vi "4.2 Arguments - Error As Arguments.vi"() -> ()   [LabVIEW 2017]
doc: "#### Overview\n\nThis example demonstrates how LabVIEW errors are passed as CSM arguments.\n\n#### Introduction\n\nThis example converts a LabVIEW error cluster into a CSM-compatible error string. This allows the CSM core parsing engine to handle LabVIEW errors from the message queue and facilitates logging internal errors. The converted error string uses the following format: `<ErrStr>[Error: error-code] error-description-As-safe-argument-string`. Additionally, `CSM - Argument Type.vi` retrieves the argument tag, which in this case is `ErrStr`.\n\n<b>Application Scenario</b>: Passing LabVIEW errors.\n\n#### Steps\n\n- Step1: Demonstrate converting an error to ErrStr and restoring it.\n- Step2: (Forward Compatibility) Demonstrate converting a previous ErrStr back to an error cluster.\n- Step3: Demonstrate converting a previous ErrStr back to an error cluster and obtaining the CSM-Argument Type."
uses:
  user.lib/_NEVSTOP/Communicable State Machine(CSM)/AdvanceAPI/CSM - Revert Arguments-Safe String.vi
  user.lib/_NEVSTOP/Communicable State Machine(CSM)/AdvanceAPI/CSM - Make String Arguments Safe.vi
  user.lib/_NEVSTOP/Communicable State Machine(CSM)/AdvanceAPI/CSM - Keywords.vi
  user.lib/_NEVSTOP/Communicable State Machine(CSM)/_Shared/Trim Single-line Text.vi
  user.lib/_NEVSTOP/Communicable State Machine(CSM)/Communicable State Machine.lvlib
  user.lib/_NEVSTOP/Communicable State Machine(CSM)/_Shared/CSM Shared.lvlib
panel:
  out "error 2":errorcluster
  out "Warning Arguments":string
  out "argument token":string
  out "<ErrStr>[Error: 472]Error String 1%0AError String 2%0AError String 3":errorcluster
  out "[Error: 502]Error String 1%0AError String 2%0AError String 3":errorcluster
  out "Error Arguments":string
  out "error":errorcluster
  # "#CSM-Example Overview\n\nThis example demonstrates how LabVIEW errors are passed as CSM arguments."
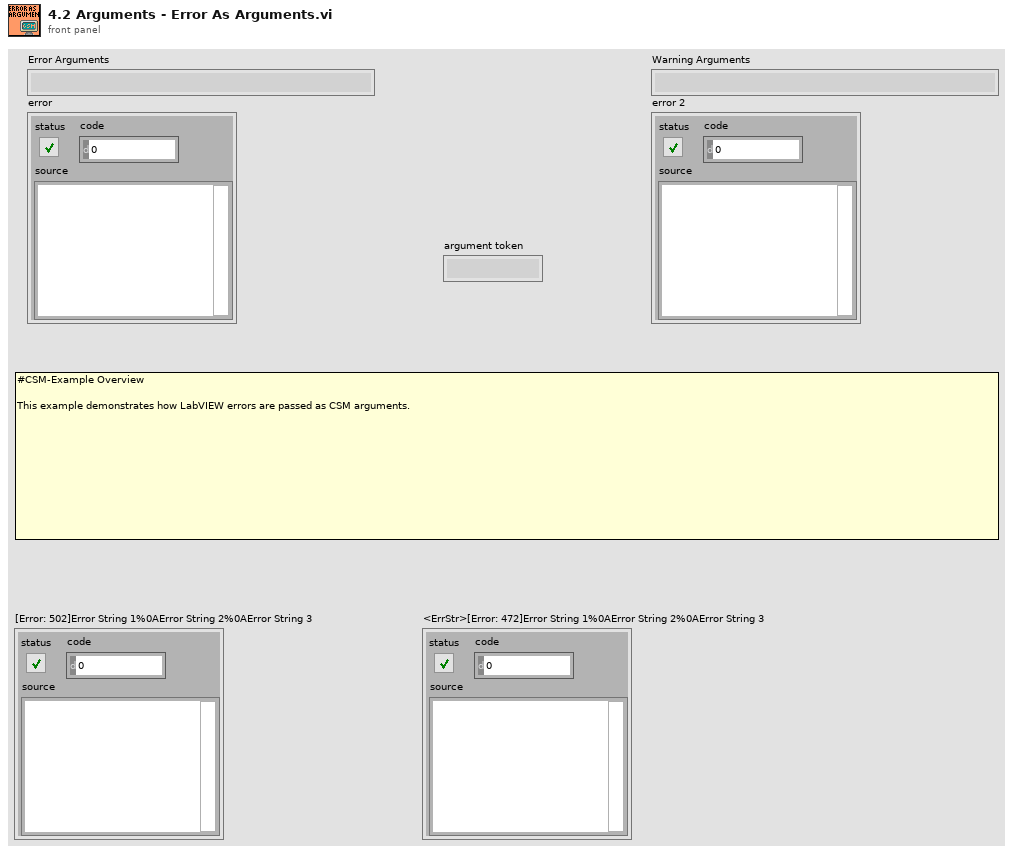
[diagram p1: front panel]
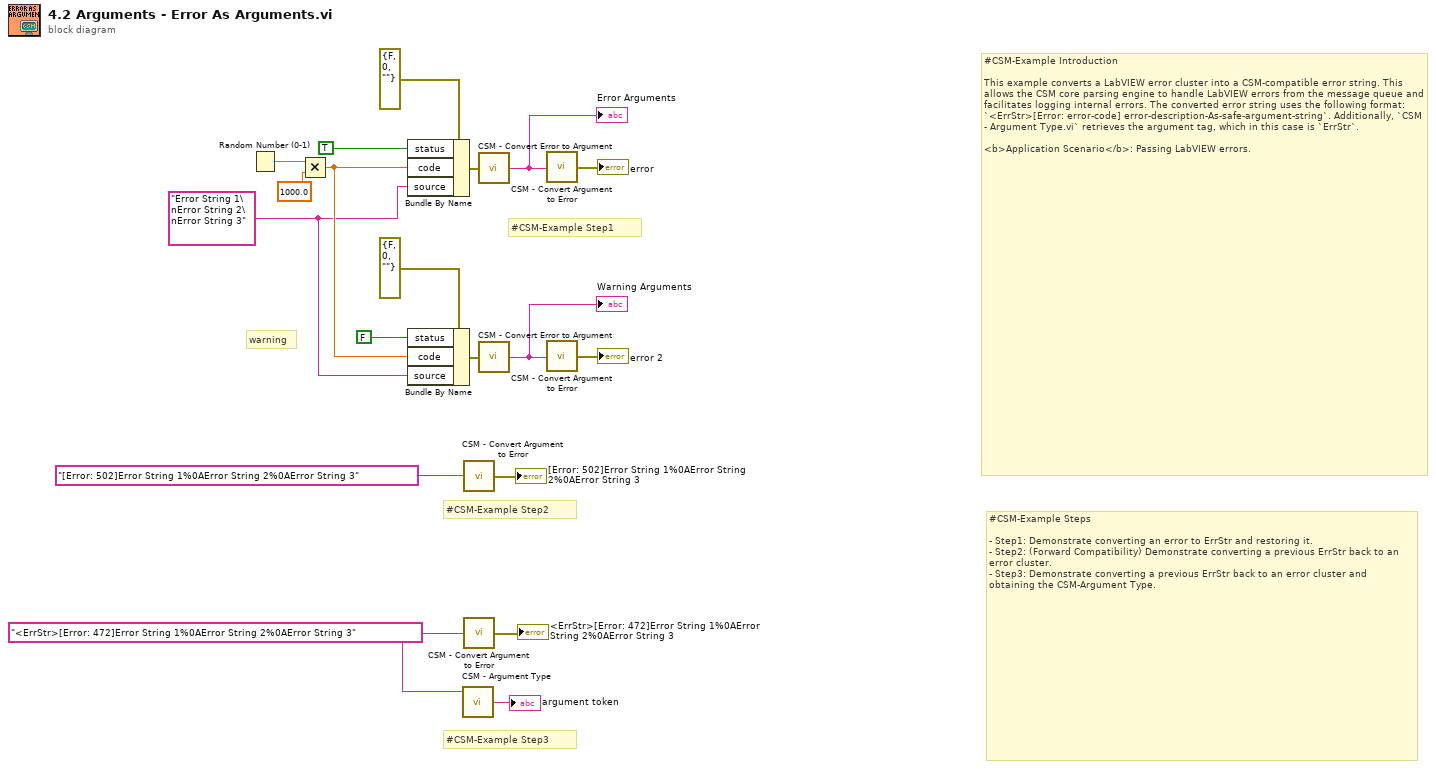
[diagram p0: block diagram]
diagram:
  w9 = "<ErrStr>[Error: 472]Error String 1%0AError String 2%0AError String 3" ("Arguments 2")
  w1 = "Error String 1\nError String 2\nError String 3" ("source")
  # "warning"
  # "#CSM-Example Step3"
  # "#CSM-Example Step2"
  # "#CSM-Example Step1"
  # "#CSM-Example Steps\n\n- Step1: Demonstrate converting an error to ErrStr and restoring it.\n- Step2: (Forward Compatibility) Demonstrate converting a previous ErrStr back to an error cluster.\n- Step3: Demonstrate converting a previous ErrStr back to an error cluster and obtaining the CSM-Argument Type."
  # "#CSM-Example Introduction\n\nThis example converts a LabVIEW error cluster into a CSM-compatible error string. This allows the CSM core parsing engine to handle LabVIEW errors from the message queue and facilitates logging internal errors. The converted error string uses the following format: `<ErrStr>[Error: error-code] error-description-As-safe-argument-string`. Additionally, `CSM - Argument Type.vi` retrieves the argument tag, which in this case is `ErrStr`.\n\n<b>Application Scenario</b>: Passing LabVIEW errors."
  n1 = Random Number (0-1)() -> (number: 0 to 1=w15:dbl)
  n2 = Multiply(x=w15, y=1000.0) -> (x*y=w2:dbl)
  n3 = Bundle By Name(cluster=errorcluster {"status"=FALSE, "code"=0, "source"=""} ("error constant"), "status"=TRUE, "code"=w2, "source"=w1) -> (w17:errorcluster)
  n4 = Bundle By Name(cluster=errorcluster {"status"=FALSE, "code"=0, "source"=""} ("error constant"), "status"=FALSE, "code"=w2, "source"=w1) -> (w5:errorcluster)
  n5 = call "CSM - Argument Type.vi"("Arguments"=w9) -> ("Argument Type"=→"argument token":string)  [unwired: 3 in, 1 out]
  n6 = call "CSM - Convert Argument to Error.vi"("Argument"="[Error: 502]Error String 1%0AError String 2%0AError String 3" ("Arguments 2")) -> ("Error"=→"[Error: 502]Error String 1%0AError String 2%0AError String 3":errorcluster)  [unwired: 4 in]
  n7 = call "CSM - Convert Argument to Error.vi"("Argument"=w9) -> ("Error"=→"<ErrStr>[Error: 472]Error String 1%0AError String 2%0AError String 3":errorcluster)  [unwired: 4 in]
  n8 = call "CSM - Convert Error to Argument.vi"("Error"=w17) -> ("Argument"=w13:string)  [unwired: 4 in]
  "Error Arguments" <- w13
  n9 = call "CSM - Convert Error to Argument.vi"("Error"=w5) -> ("Argument"=w7:string)  [unwired: 4 in]
  "Warning Arguments" <- w7
  n10 = call "CSM - Convert Argument to Error.vi"("Argument"=w13) -> ("Error"=→"error":errorcluster)  [unwired: 4 in]
  n11 = call "CSM - Convert Argument to Error.vi"("Argument"=w7) -> ("Error"=→"error 2":errorcluster)  [unwired: 4 in]
